vi "Initalize OPC UA.vi"(8 "error in (no error)":errorcluster, 11 "SM EOL Station Actor in":refnum<class "PLC Sim Controller Actor.lvclass">) -> (0 "error out":errorcluster, 3 "SM EOL Station Actor out":refnum<class "PLC Sim Controller Actor.lvclass">)   [LabVIEW 2025, in "PLC Sim Controller Actor.lvlib" / "PLC Sim Controller Actor.lvclass"]
uses:
  PLC Sim Controller Actor.lvclass
  PLC Sim Controller Actor.lvclass/PLC Sim Controller Actor.ctl
  <vilib>/OPCUA/server/Create2.vi
  <vilib>/OPCUA/NI OPC UA Server.lvlib
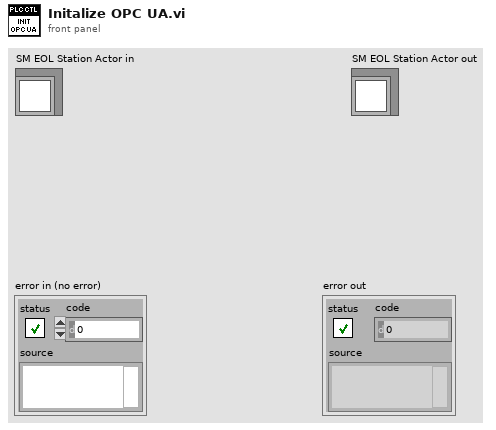
[diagram p1: front panel]
types:
  T1 = typedef "OPC UA Server Refnum.ctl" = refnum<k21>
  T2 = typedef "NodeId.ctl" = string
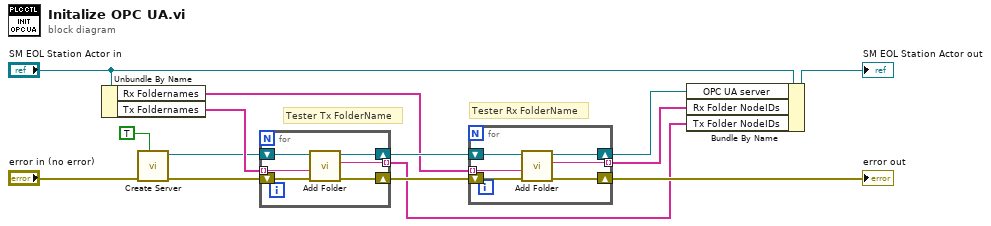
[diagram p0: block diagram]
diagram:
  # "Tester Rx FolderName"
  # "Tester Tx FolderName"
  n1 = Unbundle By Name("SM EOL Station Actor in") -> ("Rx Foldernames"=w2:string[], "Tx Foldernames"=w9:string[])
  n2 = call-poly <vilib>:"Create Server.vi"("trust all clients (F)"=TRUE, "error in (no error)"="error in (no error)") -> ("error out"=w5:errorcluster, "OPC UA server refnum out"=w4:T1)  [unwired: 7 in, 1 out]
  n3 = for {
    shift-right: [w19] -> w8
    shift-left: w5 -> [w20]
    shift-right: [w17] -> w10
    shift-left: w4 -> [w18]
    tunnel: w9 -> [w16] mode=indexing
    tunnel: [w15] -> w1 mode=indexing
    n4 = call <vilib>:"Add Folder.vi"("error in (no error)"=w20, "folder name"=w16, "OPC UA server refnum in"=w18) -> ("error out"=w19:errorcluster, "folder node ID"=w15:T2, "OPC UA server refnum out"=w17:T1)  [unwired: 5 in]
  }
  n5 = for {
    tunnel: [w25] -> w6 mode=indexing
    shift-right: [w24] -> w7
    shift-left: w10 -> [w26]
    tunnel: w2 -> [w23] mode=indexing
    shift-right: [w21] -> w13
    shift-left: w8 -> [w22]
    n6 = call <vilib>:"Add Folder.vi"("error in (no error)"=w22, "folder name"=w23, "OPC UA server refnum in"=w26) -> ("error out"=w21:errorcluster, "folder node ID"=w25:T2, "OPC UA server refnum out"=w24:T1)  [unwired: 5 in]
  }
  "error out" <- w13
  n7 = Bundle By Name(cluster="SM EOL Station Actor in", "OPC UA server"=w7, "Rx Folder NodeIDs"=w6, "Tx Folder NodeIDs"=w1) -> (→"SM EOL Station Actor out":refnum<class "PLC Sim Controller Actor.lvclass">)
